vi "PicoScope6000ExampleStreaming.vi"() -> ()   [LabVIEW 2016]
doc: "This example demonstrates how to use the PicoScope Labview library to stream data from a PicoScope 5000 Series Device"
uses:
  ps6000.dll
  ps6000Wrap.dll
panel:
  out "Device Info":T1
  in  "Trigger Settings":T2={"Trigger Enabled"=FALSE, "Trigger Source"=enum."Channel A", "Trigger Threshold (16-bit counts)"=0, "Trigger Direction"=2, "Trigger Delay (samples)"=0, "Auto Trigger Time (ms)"=1000} {"Trigger Direction" items=["Rising"=2, "Falling"=3]}
  in  "Channel A Settings":T3={"Enabled"=TRUE, "Coupling"=1, "Range"=6, "Analogue Offset"=0.0, "Bandwidth"=0} {"Bandwidth" items=["Full", "20 MHz"]; "Range" items=["10 mV", "20 mV", "50 mV", "100 mV", "200 mV", "500 mV", "1 V", "2 V", "5 V", "10 V", "20 V", "50 V ", "100 V"]; "Coupling" items=["AC", "DC 1 MOhm", "DC 50 Ohm"]}
  out "Analog Channels":T4(graph)
  out "Raw Sample Interval (sec)":dbl=1.0000000130088963e-06 format="%#.5p"
  out "Max ADC value":i16=32512
  out "Chunk time":u32
  out "Elapsed time":dbl
  in  "Poll time (ms)":u32=10 min=1 max=1000 step=1
  in  "Data file":path=path "PicoScope6000ExampleStreaming ChA Data"
  out "size(s)":i32
  out "Queue depth":i32(graph)
  out "queue depth":i32
  in  "Buffer and Transfer Settings":T5={"startIndex"=0, "Samples"=1000000, "Down Sample Ratio"=1, "Down-Sample Mode"=0} {"Down-Sample Mode" items=["None"=0, "Aggregate"=1, "Decimate"=2, "Average"=4]; "Down Sample Ratio" step=1; "Samples" format="%_6p"}
  out "TriggeredAt (In Buffer)":u32 format="%#.6p"
  out "TriggeredAt (Total samples)":u32 format="%#.6p"
  in  "Acquisition Settings":T6={"Auto Stop"=TRUE, "Desired Sample Interval"=1, "Pre-trigger Samples"=0, "Post-trigger Samples"=1000000, "Down-Sample Ratio"=1, "Down-Sample Mode"=0, "Time Units"=3} {"Time Units" items=["Nanoseconds (ns)"=2, "Microseconds (us)"=3, "Milliseconds (ms)"=4, "Seconds (s)"=5]; "Down-Sample Mode" items=["None"=0, "Aggregate"=1, "Decimate"=2, "Average"=4]; "Post-trigger Samples" format="%#.6p"; "Pre-trigger Samples" format="%#_6p"}
  out "Triggered":bool
  out "DownSample Interval (sec)":dbl=1.0000000130088963e-06 format="%#.5p"
  out "Total Samples":u32 format="%#.6p"
  out "Auto Stopped":bool
  in  "Serial Number":string
  in  "Open Using\nSerial Number":bool
  out "Number of Samples per Capture":u32 format="%#.6p"
  in  "Apply  Settings":bool
  in  "stop":bool
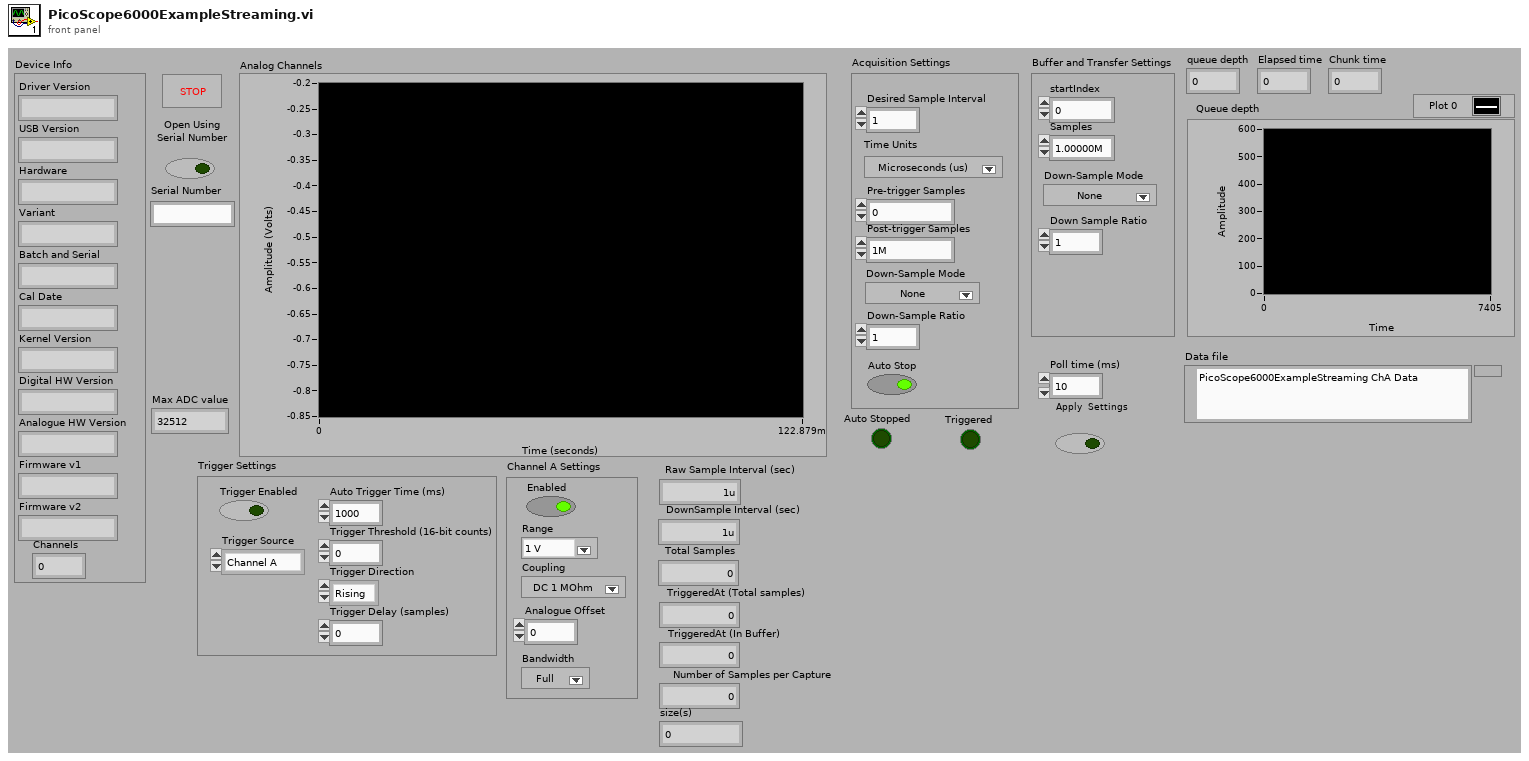
[diagram p1: front panel]
types:
  T1 = cluster{"Driver Version":string, "USB Version":string, "Hardware":string, "Variant":string, "Batch and Serial":string, "Cal Date":string, "Kernel Version":string, "Digital HW Version":string, "Analogue HW Version":string, "Firmware v1":string, "Firmware v2":string, "Channels":i16}
  T2 = cluster{"Trigger Enabled":bool, "Trigger Source":enum32{"Channel A", "Channel B", "Channel C", "Channel D", "External", "Aux."}, "Trigger Threshold (16-bit counts)":i16, "Trigger Direction":u16, "Trigger Delay (samples)":u32, "Auto Trigger Time (ms)":i16}
  T3 = cluster{"Enabled":bool, "Coupling":u32, "Range":u32, "Analogue Offset":sgl, "Bandwidth":u32}
  T4 = cluster{i32, "DownSample Interval (sec)":dbl, "Data":dbl[]}
  T5 = cluster{"startIndex":u64, "Samples":u64, "Down Sample Ratio":u64, "Down-Sample Mode":u32}
  T6 = cluster{"Auto Stop":bool, "Desired Sample Interval":u32, "Pre-trigger Samples":u32, "Post-trigger Samples":u32, "Down-Sample Ratio":u32, "Down-Sample Mode":i32, "Time Units":u32}
  T7 = enum16{"open", "open or create", "create or replace", "create", "open (read-only)"}
  T8 = cluster{"Enabled":bool, "Coupling":i32, "Range":u16, "Analogue Offset":sgl, "Bandwidth":i32}
  T9 = cluster{"Channel A Buffer":i16[], "Channel B Buffer":i16[], "Channel C Buffer":i16[], "Channel D Buffer":i16[], "Channel E Buffer":i16[], "Channel F Buffer":i16[], "Channel G Buffer":i16[], "Channel H Buffer":i16[], "Port 0":i16[], "Port 1":i16[]}
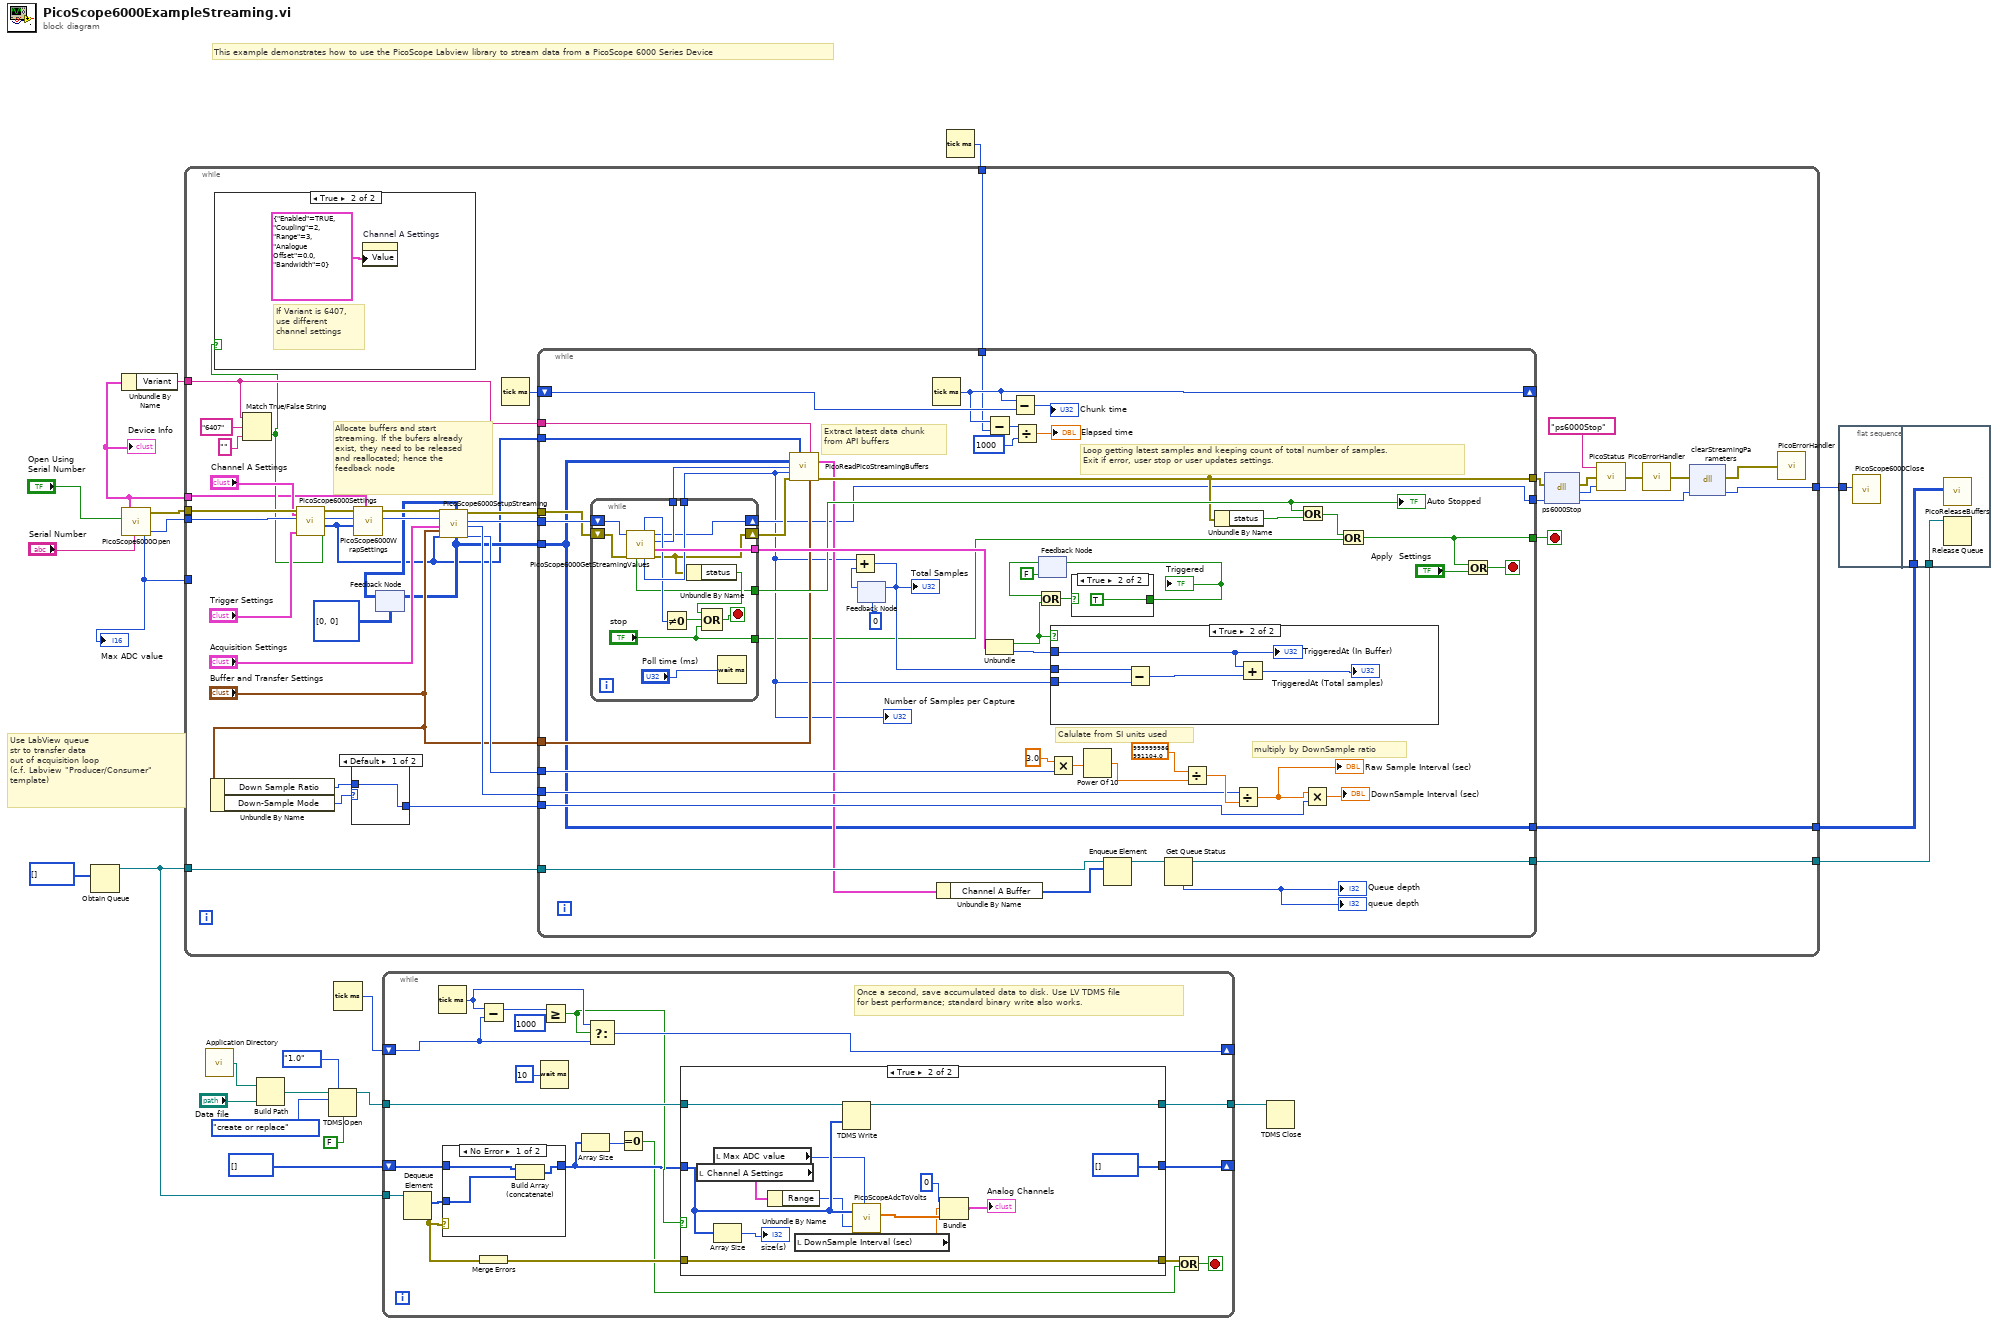
[diagram p0: block diagram]
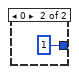
[diagram p5: hidden frame]
diagram:
  # "Use LabView queue\nstr to transfer data\nout of acquisition loop\n(c.f. Labview \"Producer/Consumer\"\ntemplate)"
  # "This example demonstrates how to use the PicoScope Labview library to stream data from a PicoScope 6000 Series Device"
  n1 = Obtain Queue(element data type=i16[] [] ("History Data")) -> (queue out=w18:refnum<queue>)  [unwired: 4 in, 2 out]
  n2 = call "PicoScope6000Open.vi"("Serial Number"="Serial Number", "Use Serial Number"="Open Using\nSerial Number") -> ("handle"=w22:i16, "Max Adc value"=w19:i16, "error out"=w23:errorcluster, "Device Info"=w1:T1)  [unwired: 1 in]
  "Max ADC value" <- w19
  "Device Info" <- w1
  n3 = Unbundle By Name(w1) -> ("Variant"=w2:string)
  n4 = call <vilib>:"Application Directory.vi"() -> ("Application Directory"=w3:path)
  n5 = Build Path(base path=w3, name or relative path="Data file") -> (appended path=w4:path)
  n6 = TDMS Open(6:FALSE ("disable buffering? (T)"), 7:enum16{"1.0", "2.0"}."1.0" ("file format version (2.0)"), 10:T7."create or replace" ("operation (0:open)"), 11:w4) -> (3:w11:refnum<k34>)  [unwired: 3 in, 1 out]
  n7 = Tick Count (ms)() -> (millisecond timer value=w13:u32)
  n8 = while {
    tunnel: w18 -> [w42]
    shift-right: [w35] -> _
    shift-left: i16[] [] ("History Data") -> [w41]
    shift-right: [w36] -> _
    shift-left: w13 -> [w37]
    tunnel: w11 -> [w34]
    tunnel: [w33] -> w10
    stop <- w27 stop-if-true
    # "Once a second, save accumulated data to disk. Use LV TDMS file\nfor best performance; standard binary write also works."
    n9 = Dequeue Element(queue=w42) -> (element=w43:i16[], error out=w32:errorcluster)  [unwired: 2 in, 2 out]
    n10 = Tick Count (ms)() -> (millisecond timer value=w38:u32)
    n11 = case shown="No Error" w32 {
      tunnel: w41 -> [w61 w62]
      tunnel: [w60 w62] -> w29
      tunnel: w43 -> [w59 _]
      frame No Error {
        n12 = Build Array (concatenate)(w61, w59) -> (w60:i16[])
      }
      frame Error {
      }
    }
    n13 = Subtract(x=w38, y=w37) -> (x-y=w40:u32)
    n14 = Merge Errors(w32) -> (w31:errorcluster)
    n15 = Wait (ms)(milliseconds to wait=u32 10) -> ()  [unwired: 1 out]
    n16 = Greater Or Equal?(x=w40, y=u32 1000) -> (x >= y?=w30:bool)
    n17 = Array Size(array=w29) -> (size(s)=w28:i32)
    n18 = Select(t=w38, s=w30, f=w37) -> (s? t:f=w36:u32)
    n19 = Equal To 0?(x=w28) -> (x = 0?=w25:bool)
    n20 = case shown="True" w30 {
      tunnel: w29 -> [w45 w54]
      tunnel: [w45 i16[] [] ("History Data")] -> w35
      tunnel: w34 -> [w44 w56]
      tunnel: [w44 w55] -> w33
      tunnel: [_ w46] -> w26
      tunnel: w31 -> [_ w46]
      frame False {
      }
      frame True {
        n21 = local read "Channel A Settings"() -> (w47:T3)
        n22 = local read "Max ADC value"() -> (w50:i16)
        n23 = Array Size(array=w54) -> (size(s)=→"size(s)":i32)
        n24 = Unbundle By Name(w47) -> ("Range"=w53:u32)
        n25 = local read "DownSample Interval (sec)"() -> (w49:dbl)
        n26 = TDMS Write(0:w56, 9:w54) -> (4:w55:refnum<k34>)  [unwired: 4 in, 3 out]
        n27 = call "PicoScopeAdcToVolts.vi"("Max_adc"=w50, "Range Index"=w53, "Data"=w54) -> ("Data"=w51:dbl[])
        n28 = Bundle(0, "DownSample Interval (sec)"=w49, "Data"=w51) -> (→"Analog Channels":T4)  [unwired: 1 in]
      }
    }
    n29 = Or(x=w26, y=w25) -> (x .or. y?=w27:bool)
  }
  n30 = Tick Count (ms)() -> (millisecond timer value=w17:u32)
  n31 = while {
    tunnel: [w70] -> w16
    tunnel: w23 -> [w102]
    tunnel: w22 -> [w103]
    tunnel: w19 -> [_]
    tunnel: [w82] -> w14
    tunnel: w18 -> [w81]
    tunnel: [w80] -> w15
    tunnel: w17 -> [w77]
    tunnel: w2 -> [w66]
    tunnel: w1 -> [w63]
    stop <- w104 stop-if-true
    # "Allocate buffers and start\nstreaming. If the bufers already\nexist, they need to be released\nand reallocated; hence the\nfeedback node"
    n32 = Unbundle By Name("Buffer and Transfer Settings") -> ("Down Sample Ratio"=w85:u64, "Down-Sample Mode"=w87:u32)
    n33 = Match True/False String(2:"" ("false string"), 3:"6407" ("true string"), 4:w66) -> (0:w65:bool)  [unwired: 1 out]
    n34 = case shown="True" w65 {
      frame False {
      }
      frame True {
        # "If Variant is 6407,\nuse different \nchannel settings"
        n35 = property on="Channel A Settings" class="Clust (strict)"("Value"=T8 {"Enabled"=TRUE, "Coupling"=2, "Range"=3, "Analogue Offset"=0.0, "Bandwidth"=0} ("Channel A Settings")) -> ()  [unwired: 2 in, 2 out]
      }
    }
    n36 = call "PicoScope6000Settings.vi"("PS6407?"=w65, "Channel A Settings"="Channel A Settings", "Trigger Settings"="Trigger Settings", "handle in"=w103, "error in"=w102) -> ("Enabled array"=w64:i16[], "handle out"=w91:i16, "error out"=w92:errorcluster)  [unwired: 4 in]
    n37 = case shown="Default" w87 {
      tunnel: [w106 u32 1 ("Down-Sample Ratio")] -> w86
      tunnel: w85 -> [w106 _]
      frame Default {
      }
      frame 0 {
      }
    }
    n38 = call "PicoScope6000WrapSettings.vi"("Device Info"=w63, "enabledChannels"=w64, "Handle In"=w91, "error in (no error)"=w92) -> ("Handle Out"=w94:i16, "error out"=w93:errorcluster)  [unwired: 6 in]
    n39 = feedback #1(u64[][] [[0], [0]] ("Pointer array")) -> (w79:u64[][])
    n40 = call "PicoScope6000SetupStreaming.vi"("error in"=w93, "handle in"=w94, "Acquisition Settings"="Acquisition Settings", "Buffer and Transfer Settings"="Buffer and Transfer Settings", "enabled array"=w64, "Pointers In"=w79) -> ("Pointer array"=w76:u64[][], "error out"=w100:errorcluster, "handle out"=w101:i16, "Sample Interval"=w90:u32, "sampleIntervalTimeUnits"=w89:u32)  [unwired: 9 in]
    n41 = feedback-in #1(w76) -> ()
    n42 = Tick Count (ms)() -> (millisecond timer value=w78:u32)
    n43 = while {
      tunnel: [w114] -> w99
      tunnel: [w157] -> w104
      tunnel: w101 -> [w133]
      tunnel: w100 -> [w132]
      tunnel: w90 -> [w136]
      tunnel: w89 -> [w144]
      tunnel: [w129] -> w88
      tunnel: w86 -> [w134]
      tunnel: "Buffer and Transfer Settings" -> [w131]
      tunnel: w64 -> [w128]
      tunnel: [w126] -> w82
      tunnel: w81 -> [w124]
      tunnel: w76 -> [w122]
      tunnel: [w122] -> w80
      shift-right: [w117] -> _
      shift-left: w78 -> [w118]
      tunnel: w77 -> [w116]
      tunnel: w66 -> [w111]
      stop <- w156 stop-if-true
      # "Loop getting latest samples and keeping count of total number of samples. \nExit if error, user stop or user updates settings."
      # "Extract latest data chunk\nfrom API buffers"
      # "Calulate from SI units used"
      # "multiply by DownSample ratio"
      n44 = while {
        tunnel: [w172] -> w155
        tunnel: [w164] -> w152
        tunnel: [w163] -> w113
        tunnel: [w171] -> w112
        shift-right: [w162] -> w114
        shift-left: w133 -> [w161]
        shift-right: [w159] -> w130
        shift-left: w132 -> [w160]
        tunnel: ["stop"] -> w109
        stop <- w166 stop-if-true
        n45 = call "PicoScope6000GetStreamingValues.vi"("error in"=w160, "handle in"=w161) -> ("error out"=w159:errorcluster, "Trigger"=w172:cluster{bool, "triggeredAt":u32}, "Start Index"=w163:u32, "handle out"=w162:i16, "Number of Samples"=w171:u32, "ready"=w169:i16, "Auto Stopped"=w164:bool)  [unwired: 3 in]
        n46 = Not Equal To 0?(x=w169) -> (x != 0?=w167:bool)
        n47 = Unbundle By Name(w159) -> ("status"=w168:bool)
        n48 = Compound Arithmetic op=OR(w168, w167, "stop") -> (w166:bool)
        n49 = Wait (ms)(milliseconds to wait="Poll time (ms)") -> ()  [unwired: 1 out]
      }
      "Number of Samples per Capture" <- w112
      "Auto Stopped" <- w152
      n50 = call "PicoReadPicoStreamingBuffers.vi"("enabled array"=w128, "Buffer and Transfer Settings"=w131, "Variant"=w111, "Pointer array"=w122, "Offset Index"=w113, "Number of Samples"=w112, "error in (no error)"=w130) -> ("Buffers (Max or non-aggregated)"=w123:T9, "error out"=w129:errorcluster)  [unwired: 6 in, 1 out]
      n51 = feedback #2(u32 0) -> (w148:u32)
      n52 = Add(x=w112, y=w148) -> (x+y=w140:u32)
      "Total Samples" <- w140
      n53 = feedback-in #2(w140) -> ()
      n54 = Tick Count (ms)() -> (millisecond timer value=w117:u32)
      n55 = Unbundle By Name(w123) -> ("Channel A Buffer"=w108:i16[])
      n56 = Subtract(x=w117, y=w116) -> (x-y=w121:u32)
      n57 = Unbundle(w155) -> (w138:bool, "triggeredAt"=w137:u32)
      n58 = Subtract(x=w117, y=w118) -> (x-y=→"Chunk time":u32)
      n59 = Divide(x=w121, y=u32 1000) -> (x/y=→"Elapsed time":dbl)
      n60 = feedback #3(FALSE) -> (w150:bool)
      n61 = Or(x=w150, y=w138) -> (x .or. y?=w141:bool)
      n62 = Multiply(x=3.0, y=w144) -> (x*y=w142:dbl)
      n63 = case shown="True" w138 {
        tunnel: w112 -> [_ w173]
        tunnel: w140 -> [_ w177]
        tunnel: w137 -> [_ w175]
        frame False {
        }
        frame True {
          n64 = Subtract(x=w177, y=w173) -> (x-y=w176:u32)
          n65 = Add(x=w175, y=w176) -> (x+y=→"TriggeredAt (Total samples)":u32)
          "TriggeredAt (In Buffer)" <- w175
        }
      }
      n66 = case shown="True" w141 {
        selector: w141 -> [w178 _]
        tunnel: [w178 TRUE] -> w139
        frame False {
        }
        frame True {
        }
      }
      "Triggered" <- w139
      n67 = feedback-in #3(w139) -> ()
      n68 = Power Of 10(x=w142) -> (10^x=w143:dbl)
      n69 = Enqueue Element(queue=w124, element=w108) -> (queue out=w125:refnum<queue>)  [unwired: 2 in, 2 out]
      n70 = Get Queue Status(queue=w125) -> (queue out=w126:refnum<queue>, # elements in queue=→"queue depth" →"Queue depth":i32)  [unwired: 2 in, 6 out]
      n71 = Divide(x=sgl 1000000000000000.0 ("y"), y=w143) -> (x/y=w145:dbl)
      n72 = Unbundle By Name(w129) -> ("status"=w154:bool)
      n73 = Divide(x=w136, y=w145) -> (x/y=w110:dbl)
      "Raw Sample Interval (sec)" <- w110
      n74 = Or(x=w152, y=w154) -> (x .or. y?=w153:bool)
      n75 = Multiply(x=w110, y=w134) -> (x*y=→"DownSample Interval (sec)":dbl)
      n76 = Or(x=w153, y=w109) -> (x .or. y?=w157:bool)
      n77 = Or(x=w157, y="Apply  Settings") -> (x .or. y?=w156:bool)
    }
    n78 = dll-call lib="ps6000.dll" fn="ps6000Stop"(error in=w88, "handle"=w99) -> (error out=w97:errorcluster, "PICO_STATUS"=w98:u32, "handle"=w71:i16)  [unwired: 2 in, 1 out]
    n79 = call "PicoStatus.vi"("PICO STATUS"=w98, "error in"=w97, "source"="ps6000Stop") -> ("error out"=w96:errorcluster)
    n80 = call "PicoErrorHandler.vi"("error in"=w96) -> ("error out"=w72:errorcluster)
    n81 = dll-call lib="ps6000Wrap.dll" fn="clearStreamingParameters"(error in=w72, "handle"=w71) -> (error out=w69:errorcluster, "handle"=w70:i16)  [unwired: 3 in, 1 out]
    n82 = call "PicoErrorHandler.vi"("error in"=w69) -> ()  [unwired: 1 out]
  }
  n83 = TDMS Close(11:w10) -> ()  [unwired: 1 in, 2 out]
  n84 = flat-sequence {
    tunnel: w16 -> [w180]
    tunnel: w15 -> [w182]
    tunnel: w14 -> [w181]
    frame #0 {
      n85 = call "PicoScope6000Close.vi"("handle"=w180) -> ()
    }
    frame #1 {
      n86 = call "PicoReleaseBuffers.vi"("Pointer array"=w182) -> ()  [unwired: 10 in, 1 out]
      n87 = Release Queue(queue=w181) -> ()  [unwired: 2 in, 3 out]
    }
  }
